vi "Stream Create.vi"   [LabVIEW 2020, in "OpenLvVision_OpenCv.lvlib" / "Cuda.lvlib" / "Stream.lvclass"]
doc: "Object by Reference!\nCreates and initializes a new CUDA Stream. \nA stream represents a dedicated, asynchronous execution queue."
uses:
  Stream.lvclass
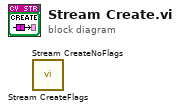
[diagram p0: block diagram]
diagram:
  n1 = call "Stream CreateFlags.vi"() -> ()  [unwired: 10 in, 2 out]
  n2 = call "Stream CreateNoFlags.vi"() -> ()  [unwired: 10 in, 2 out]
